vi "Write outputFolder.vi"(8 "error in (no error)":errorcluster, 10 "outputFolder":path, 11 "ZM-CP-FL-file_logger in":refnum<class "ZM-CP-FL-file_logger.lvclass">) -> (0 "error out":errorcluster, 3 "ZM-CP-FL-file_logger out":refnum<class "ZM-CP-FL-file_logger.lvclass">)   [LabVIEW 2020, in "ZM-CP-FL-file_logger.lvlib" / "ZM-CP-FL-file_logger.lvclass"]
doc: "Writes one field of this class's private data. Generated by lvai_create_accessors from the class private data control."
uses:
  ZM-CP-FL-file_logger.lvclass
  ZM-CP-FL-file_logger.lvclass/ZM-CP-FL-file_logger.ctl
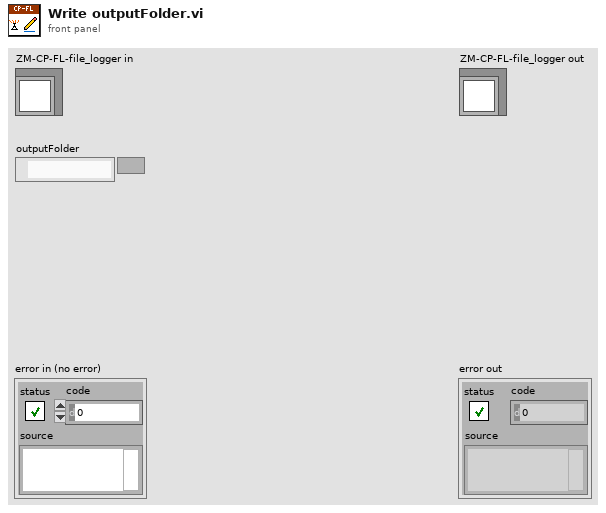
[diagram p1: front panel]
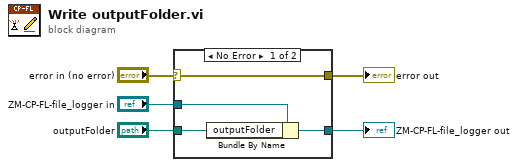
[diagram p0: block diagram]
diagram:
  n1 = case shown="No Error" "error in (no error)" {
    selector: "error in (no error)" -> [w9 w10]
    tunnel: [w9 w10] -> w4
    tunnel: [w7 w11] -> w2
    tunnel: "ZM-CP-FL-file_logger in" -> [w8 w11]
    tunnel: "outputFolder" -> [w6 _]
    frame No Error {
      n2 = Bundle By Name(cluster=w8, "outputFolder"=w6) -> (w7:refnum<class "ZM-CP-FL-file_logger.lvclass">)
    }
    frame Error {
    }
  }
  "error out" <- w4
  "ZM-CP-FL-file_logger out" <- w2
